vi "VI Tree - Caraya.vi"   [LabVIEW 2020]
doc: "Simplified VI Tree of the public supported methods of Caraya Unit Test Framework"
uses:
  classes/Assert/Assert False.vi
  classes/Assert/Assert True.vi
  run-tests/Run Test (Scalar Path).vi
  run-tests/Run Test (VIRefnum Scalar).vi
  run-tests/Run Test (Array Path).vi
  run-tests/Run Test (VIRefnum Array).vi
  run-tests/Run Test (ProjectRefnum).vi
  run-tests/Run Test (Object Array).vi
  run-tests/Run Test (Object).vi
  run-tests/Run Test (LibraryRefnum).vi
  classes/Assert/Assert.lvclass
  Caraya.lvlib
  classes/Test/Test.lvclass
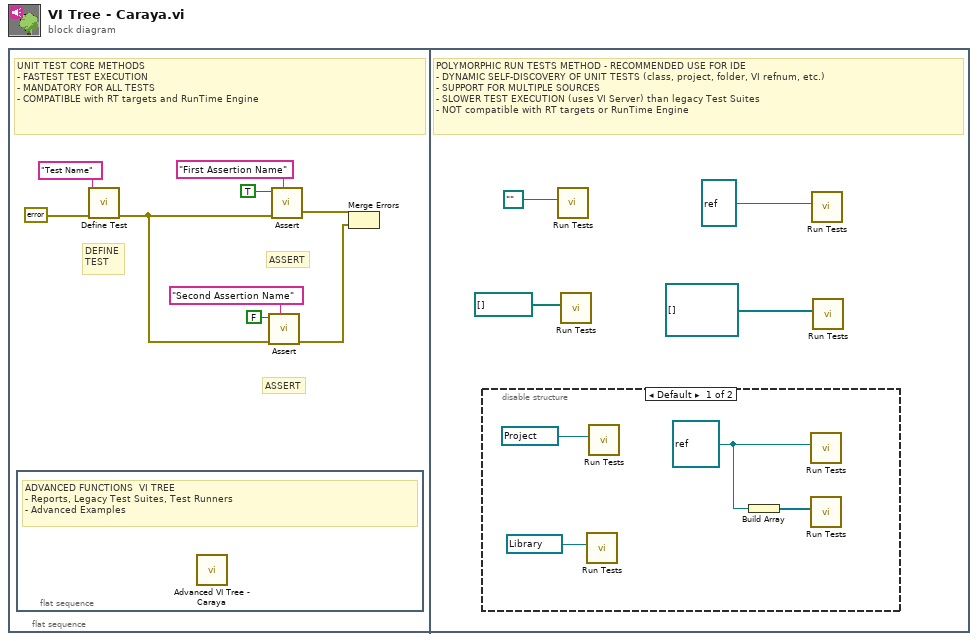
[diagram p0: block diagram]
diagram:
  n1 = flat-sequence {
    frame #0 {
      # "ASSERT"
      # "ASSERT"
      # "DEFINE\nTEST"
      # "UNIT TEST CORE METHODS\n- FASTEST TEST EXECUTION\n- MANDATORY FOR ALL TESTS\n- COMPATIBLE with RT targets and RunTime Engine"
      n2 = flat-sequence {
        frame #0 {
          # "ADVANCED FUNCTIONS  VI TREE\n- Reports, Legacy Test Suites, Test Runners\n- Advanced Examples"
          n3 = call "Advanced VI Tree - Caraya.vi"() -> ()  [unwired: 1 in]
        }
      }
      n4 = call "Define Test.vi"("error in (no error)"=errorcluster {"status"=FALSE, "code"=0, "source"=""}, "Label (VI Title)"="Test Name") -> ("error out"=w4:errorcluster)  [unwired: 8 in, 1 out]
      n5 = call-poly "Assert.vi"("Label"="Second Assertion Name" ("Label (VI Title)"), "error in (no error)"=w4, "False?"=FALSE) -> ("error out"=w3:errorcluster)  [unwired: 7 in, 1 out]
      n6 = call-poly "Assert.vi"("Label"="First Assertion Name" ("Label (VI Title)"), "error in (no error)"=w4, "True?"=TRUE) -> ("error out"=w5:errorcluster)  [unwired: 7 in, 1 out]
      n7 = Merge Errors(w5, w3) -> ()  [unwired: 1 out]
    }
    frame #1 {
      # "POLYMORPHIC RUN TESTS METHOD - RECOMMENDED USE FOR IDE\n- DYNAMIC SELF-DISCOVERY OF UNIT TESTS (class, project, folder, VI refnum, etc.)\n- SUPPORT FOR MULTIPLE SOURCES\n- SLOWER TEST EXECUTION (uses VI Server) than legacy Test Suites\n- NOT compatible with RT targets or RunTime Engine"
      n8 = disable-structure shown="Default" {
        frame condition #0 (active) {
          w15 = refnum<class> refnum ("Object")
          n9 = call-poly "Run Tests.vi"("Library Refnum"=refnum<vi> refnum) -> ()  [unwired: 9 in, 2 out]
          n10 = call-poly "Run Tests.vi"("Project Refnum"=refnum<vi> refnum) -> ()  [unwired: 9 in, 2 out]
          n11 = Build Array(w15) -> (w16:refnum<class>[])
          n12 = call-poly "Run Tests.vi"("Object"=w15) -> ()  [unwired: 9 in, 2 out]
          n13 = call-poly "Run Tests.vi"("Objects"=w16) -> ()  [unwired: 9 in, 2 out]
        }
        frame condition #1 {
        }
      }
      n14 = call-poly "Run Tests.vi"("Test Path"=path "") -> ()  [unwired: 9 in, 2 out]
      n15 = call-poly "Run Tests.vi"("Paths"=path[] []) -> ()  [unwired: 9 in, 2 out]
      n16 = call-poly "Run Tests.vi"("VI Refnum"=refnum<vi> refnum) -> ()  [unwired: 9 in, 2 out]
      n17 = call-poly "Run Tests.vi"("VI Refnums"=refnum<vi>[] []) -> ()  [unwired: 9 in, 2 out]
    }
  }
